vi "VIH - CHM Project - Write TOC File.vi"(8 "error in":errorcluster, 9 "Project Files":T2, 10 "Target TOC File":path, 11 "Template TOC File":path) -> (0 "error out":errorcluster)   [LabVIEW 2014]
doc: "::: VI Helpeks :::\nCopyright (c) 2000-2026 Konstantin Shifershteyn. All rights reserved."
uses:
  _VIH HelpGen - Palette.llb/VIH HelpGen Typedef - Palette - Item Type Enum.ctl
panel:
  # "VI Helpeks\nCopyright (c) 2012-2026 Konstantin Shifershteyn"
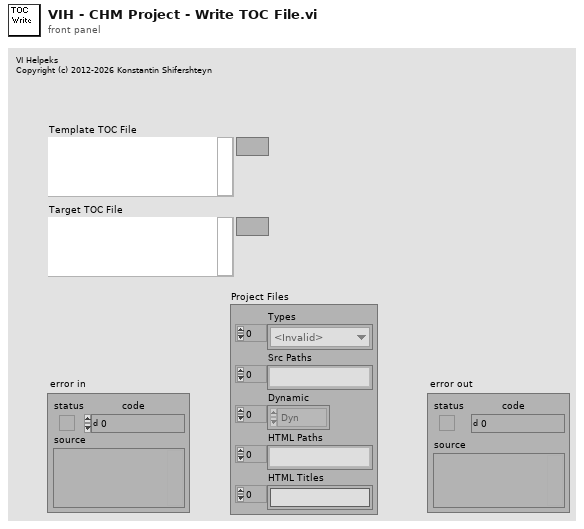
[diagram p1: front panel]
types:
  T1 = typedef "VIH HelpGen Typedef - Palette - Item Type Enum.ctl" = enum32{"<Invalid>", "<unknown>", "VI", "Menu", "LV Func", "Express VI", "Poly VI", "CTL", "HTML"}
  T2 = cluster{"Types":T1[], "Src Paths":path[], "Dynamic":enum16{"Dyn", "Stat", "Both"}[], "HTML Paths":path[], "HTML Titles":string[]}
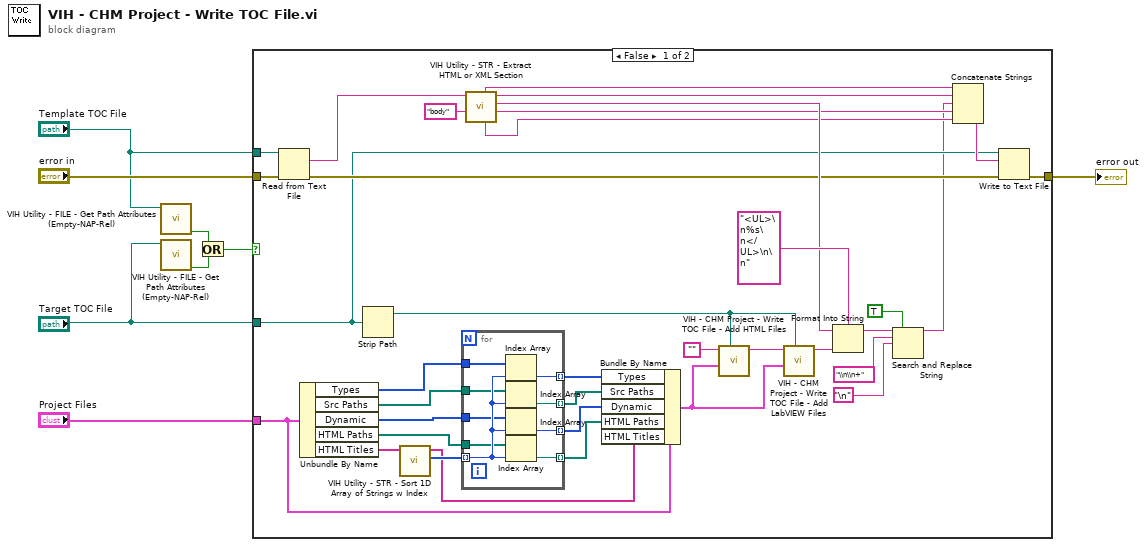
[diagram p0: block diagram]
diagram:
  n1 = call "VIH Utility - FILE - Get Path Attributes (Empty-NAP-Rel).vi"("Path"="Template TOC File") -> ("Not A Path or Empty path"=w3:bool)  [unwired: 6 in, 4 out]
  n2 = call "VIH Utility - FILE - Get Path Attributes (Empty-NAP-Rel).vi"("Path"="Target TOC File") -> ("Not A Path or Empty path"=w2:bool)  [unwired: 6 in, 4 out]
  n3 = Or(x=w3, y=w2) -> (x .or. y?=w1:bool)
  n4 = case shown="False" w1 {
    tunnel: "Template TOC File" -> [w43 _]
    tunnel: "error in" -> [w42 w54]
    tunnel: [w33 w54] -> w7
    tunnel: "Target TOC File" -> [w32 _]
    tunnel: "Project Files" -> [w20 _]
    frame False {
      n5 = Read from Text File(file (use dialog)=w43, error in=w42) -> (text=w41:string, error out=w35:errorcluster)  [unwired: 2 in, 2 out]
      n6 = Unbundle By Name(w20) -> ("Types"=w21:T1[], "Src Paths"=w22:path[], "Dynamic"=w23:enum16{"Dyn", "Stat", "Both"}[], "HTML Paths"=w24:path[], "HTML Titles"=w26:string[])
      n7 = Strip Path(path=w32) -> (stripped path=w29:path)  [unwired: 1 out]
      n8 = call "VIH Utility - STR - Sort 1D Array of Strings w Index.vi"("Array in"=w26) -> ("Index array"=w25:i32[], "Array out"=w15:string[])  [unwired: 7 in, 2 out]
      n9 = for {
        tunnel: w25 -> [w53] mode=indexing
        tunnel: w24 -> [w52]
        tunnel: w23 -> [w51]
        tunnel: w22 -> [w50]
        tunnel: w21 -> [w49]
        tunnel: [w48] -> w19 mode=indexing
        tunnel: [w47] -> w18 mode=indexing
        tunnel: [w46] -> w17 mode=indexing
        tunnel: [w45] -> w16 mode=indexing
        n10 = Index Array(array=w49, index=w53) -> (element=w48:T1)
        n11 = Index Array(array=w50, index=w53) -> (element=w47:path)
        n12 = Index Array(array=w51, index=w53) -> (element=w46:enum16{"Dyn", "Stat", "Both"})
        n13 = Index Array(array=w52, index=w53) -> (element=w45:path)
      }
      n14 = call "VIH Utility - STR - Extract HTML or XML Section.vi"("Section name"="body", "HTML in"=w41) -> ("end"=w36:string, "body"=w39:string, "start"=w37:string, "after"=w31:string, "before"=w38:string)  [unwired: 5 in]
      n15 = Bundle By Name(cluster=w20, "Types"=w19, "Src Paths"=w18, "Dynamic"=w17, "HTML Paths"=w16, "HTML Titles"=w15) -> (w14:T2)
      n16 = call "VIH - CHM Project - Write TOC File - Add HTML Files.vi"("Base Dir Path"=w29, "Project Files"=w14, "HTML in"="") -> ("HTML out"=w30:string)  [unwired: 7 in, 1 out]
      n17 = call "VIH - CHM Project - Write TOC File - Add LabVIEW Files.vi"("Base Dir Path"=w29, "Project Files"=w14, "HTML in"=w30) -> ("HTML out"=w27:string)  [unwired: 7 in, 1 out]
      n18 = Format Into String(format string="<UL>\n%s\n</UL>\n\n", initial string=w39, w27) -> (resulting string=w13:string)  [unwired: 1 in, 1 out]
      n19 = Search and Replace String(replace all?=TRUE, input string=w13, search string="\\n\\n+", replace string="\n") -> (result string=w9:string)  [unwired: 4 in, 3 out]
      n20 = Concatenate Strings(w38, w37, w9, w36, w31) -> (w34:string)
      n21 = Write to Text File(file (use dialog)=w32, text=w34, error in=w35) -> (error out=w33:errorcluster)  [unwired: 1 in, 2 out]
    }
    frame True {
    }
  }
  "error out" <- w7
